vi "CRIOUI.vi"() -> ()   [LabVIEW 2014, in "PLTarget cRIO.lvclass"]
uses:
  PLTarget cRIO.lvclass
  <vilib>/NI/Tag Bus Module Framework/root configuration/Target Types.ctl
  <vilib>/NI/Configuration Framework/Node/NodeRef.ctl
  <vilib>/NI/Configuration Framework/Node/NISE_CEF_Node.lvclass
  <vilib>/NI/AMC/Message Queue.ctl
  <vilib>/NI/AMC/Message.ctl
  <vilib>/NI/Tools/Keyed Array/KeyedArray.ctl
  <vilib>/NI/Configuration Framework/Node/UserEventRef.ctl
  <vilib>/NI/Configuration Framework/Controls/EventCluster.ctl
  <vilib>/NI/Configuration Framework/Node/RefreshUIEvent.ctl
  <vilib>/NI/Configuration Framework/Node/CacheState.ctl
  <vilib>/NI/Configuration Framework/Node/StopEvent.ctl
  <vilib>/NI/Configuration Framework/Node/NodeChangeEvent.ctl
  Configuration Editor/subVIs/Additional Files Array.ctl
  Configuration Editor/Classes/TBM Configuration Node/deployment configuration.ctl
  <vilib>/Utility/miscctls.llb/LVPositionTypeDef.ctl
  Configuration Editor/Classes/Targets/Targets.lvclass/Targets.ctl
  PLTarget cRIO.lvclass/PLTarget cRIO.ctl
  Framework Configuration Classes/target configuration/PL_Target Configuration.lvclass/PL_Target Configuration.ctl
  <vilib>/NI/Configuration Framework/serializable node/NISE_CEF_serializable node.lvclass
  <vilib>/NI/Tag Bus Module Framework/root configuration/TBM configuration.lvclass
  Configuration Editor/Classes/Targets/Write additional files.vi
  Configuration Editor/Classes/Targets/Read additional files.vi
  <vilib>/NI/Configuration Framework/serializable configuration/set alias.vi
  <vilib>/NI/Configuration Framework/serializable configuration/get alias.vi
  <vilib>/NI/Configuration Framework/serializable configuration/NISE_CEF_serializable configuration.lvclass
  Framework Configuration Classes/target configuration/PL_Target Configuration.lvclass
  Configuration Editor/Classes/Targets/Targets.lvclass
  <vilib>/NI/DCAF UI Toolkit/Controls/DCAF UI Elements.lvlib
  <vilib>/NI/Tools/Keyed Array/Tools_KeyedArray.lvlib
  <vilib>/NI/AMC/AMC.lvlib
  <vilib>/NI/Configuration Framework/NISE_CEF_TreeControl.lvlib
  Configuration Editor/Classes/TBM Configuration Node/TBM Configuration Node.lvclass
panel:
  in  "Top Level Tab Control":enum32{"Configuration", "Additional Files"}(tab)
  in  "Target Type":T1=enum."Linux RT ARM"
  in  "IP":string
  in  "Name":string
  in  "Includes file path":path
  in  "path to deploy on target relative to root (c:\\ or /home/lvuser/)":path
  in  "generate includes file":bool
  in  "load bitfile":bool
  in  "RIO FPGA":string="RIO0"
  in  "bitfile path on target relative to root (c:\\ or /home/lvuser/)":path
  in  "Local Bitfile Path":path
  in  "Additional Files":T2
  in  "node change":T4
  in  "stop event":T5
  in  "cache state":T6
  in  "refresh UI":T7
  in  "open fp?":bool=TRUE
  in  "user event":T8
  in  "main queue":T9
  in  "node ref":T10
  # "Target Information"
  # "Deployment Settings"
  # "FPGA Settings"
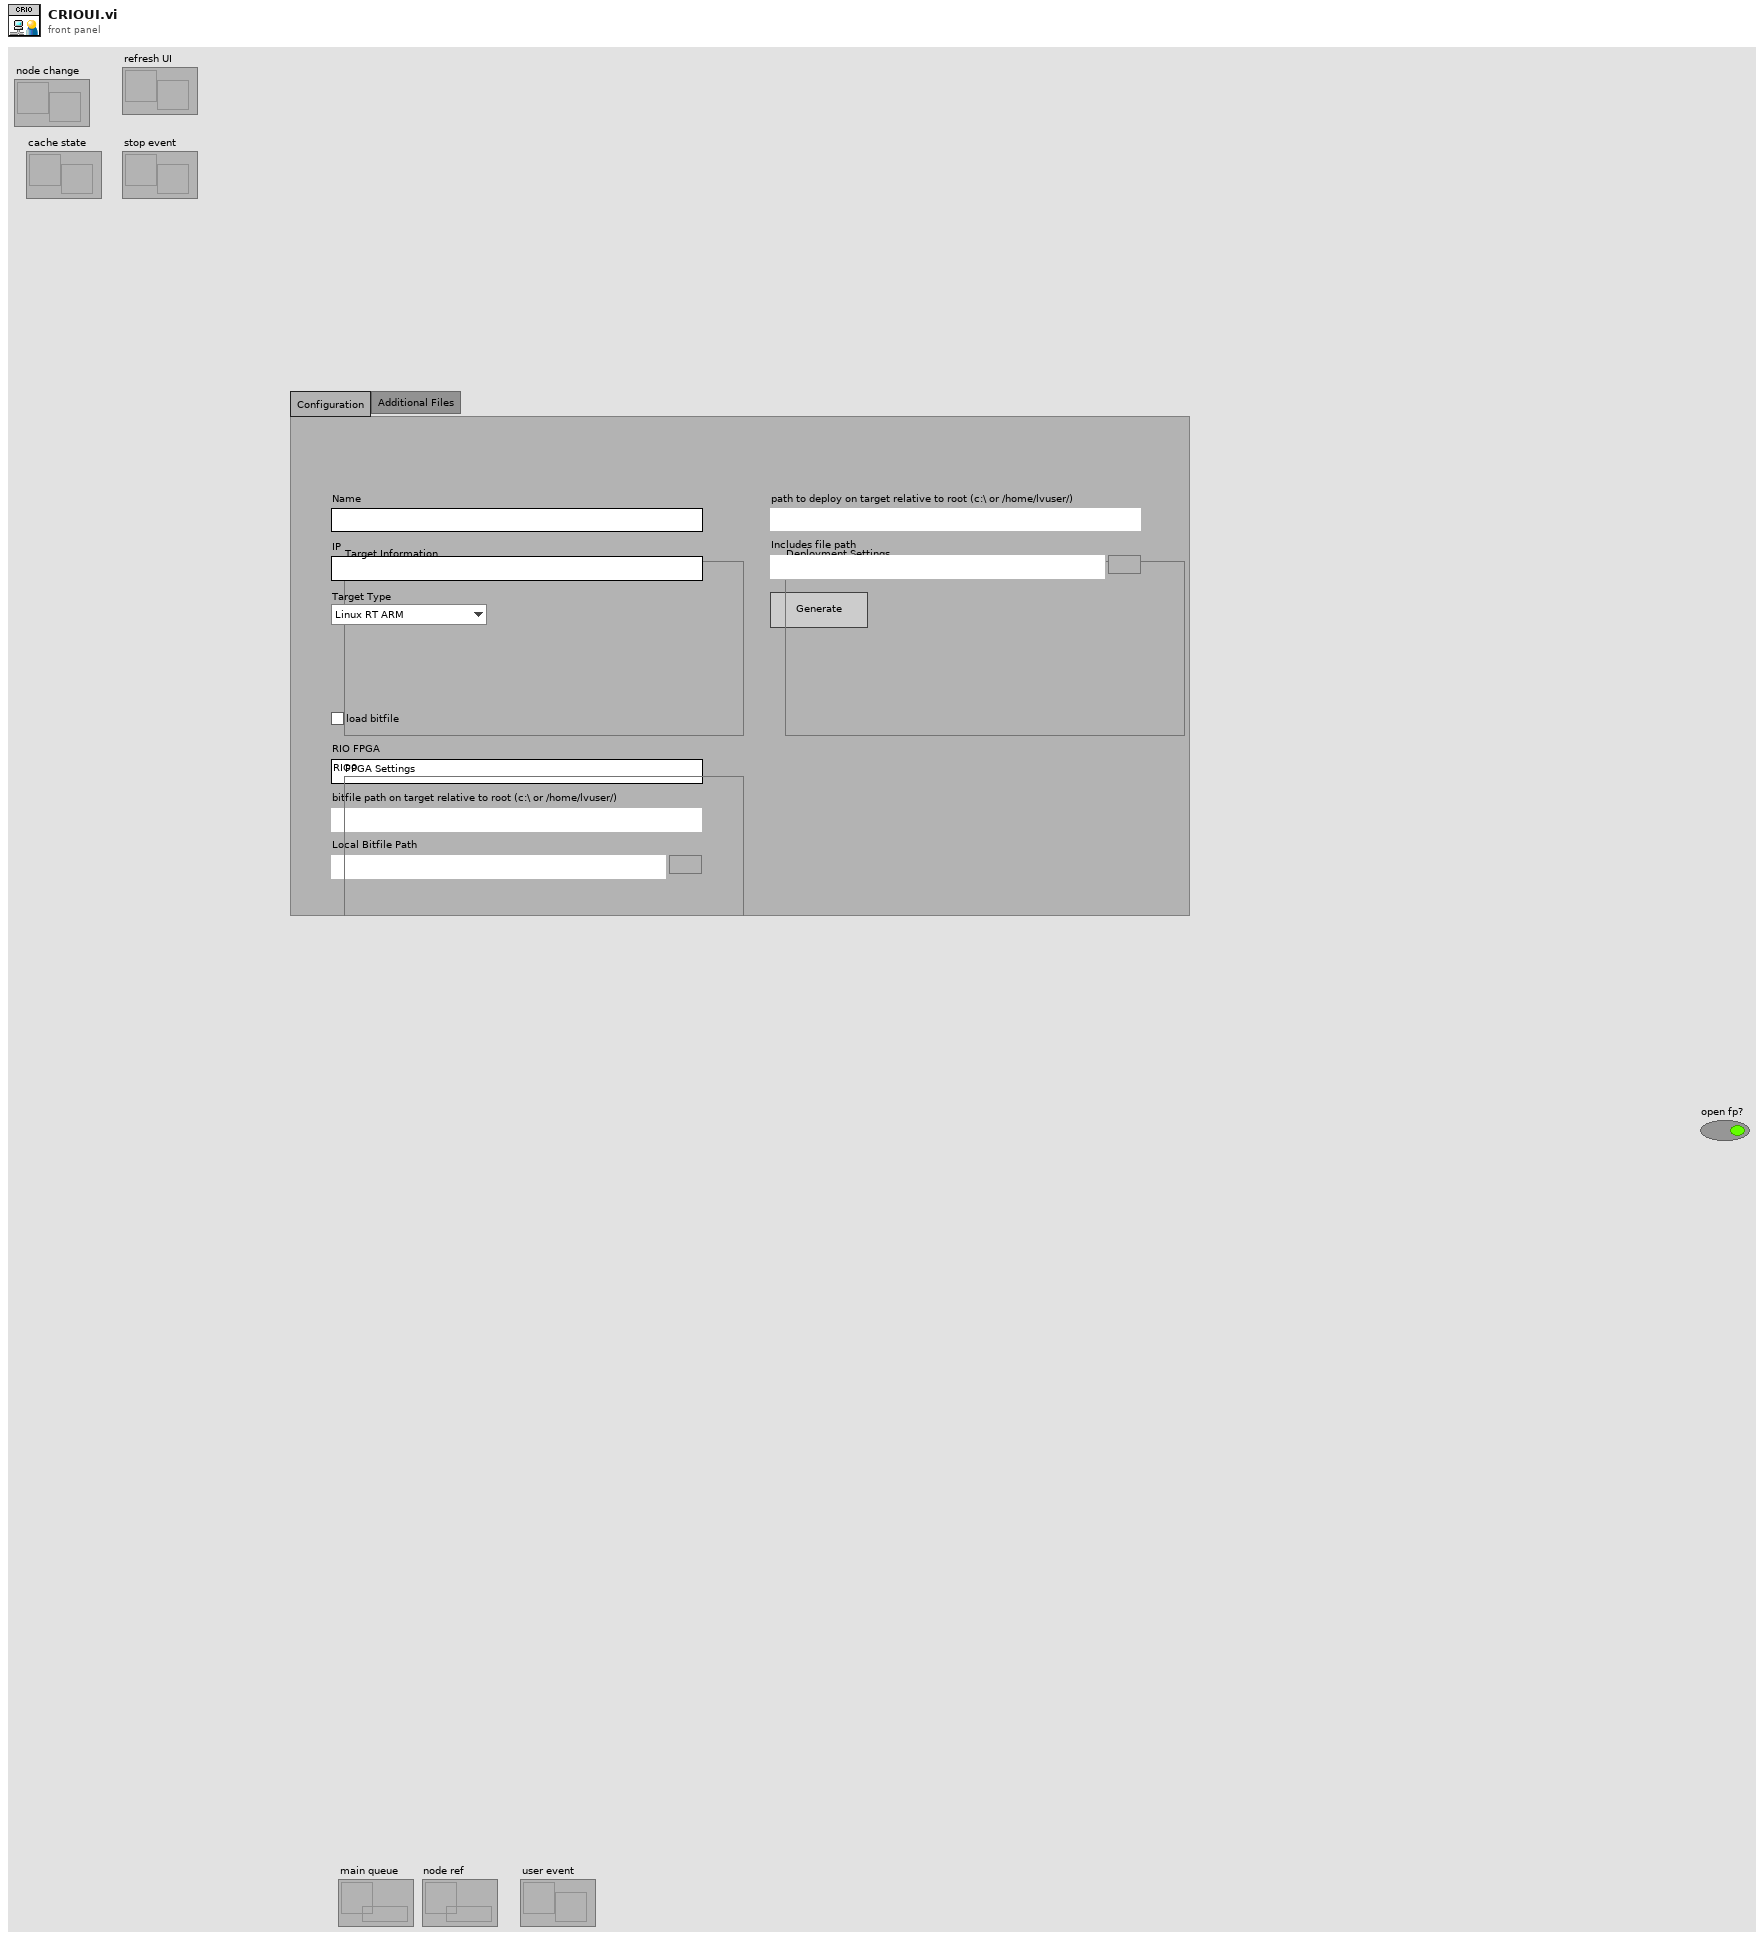
[diagram p1: front panel]
types:
  T1 = typedef "TBM configuration.lvclass/Target Types.ctl" = enum16{"Windows", "Mac", "Linux", "Linux RT ARM", "VxWorks", "Pharlap", "Other", "Linux RT x64"}
  T2 = typedef "Additional Files Array.ctl" = T3[]
  T3 = typedef "PL Framework Configuration Tool.lvlib/TBM Configuration Node.lvclass/deployment configuration.ctl" = cluster{"local path":path, "remote path (relative to root)":path}
  T4 = typedef "NISE_CEF_Node.lvclass/NodeChangeEvent.ctl" = refnum<user-event>
  T5 = typedef "NISE_CEF_Node.lvclass/StopEvent.ctl" = refnum<user-event>
  T6 = typedef "NISE_CEF_Node.lvclass/CacheState.ctl" = refnum<user-event>
  T7 = typedef "NISE_CEF_Node.lvclass/RefreshUIEvent.ctl" = refnum<user-event>
  T8 = typedef "NISE_CEF_Node.lvclass/UserEventRef.ctl" = refnum<user-event>
  T9 = typedef "AMC.lvlib/Message Queue.ctl" = refnum<queue>
  T10 = typedef "NISE_CEF_Node.lvclass/NodeRef.ctl" = refnum<data-value>
  T11 = typedef "LVPositionTypeDef.ctl" = cluster{"Left":i32, "Top":i32}
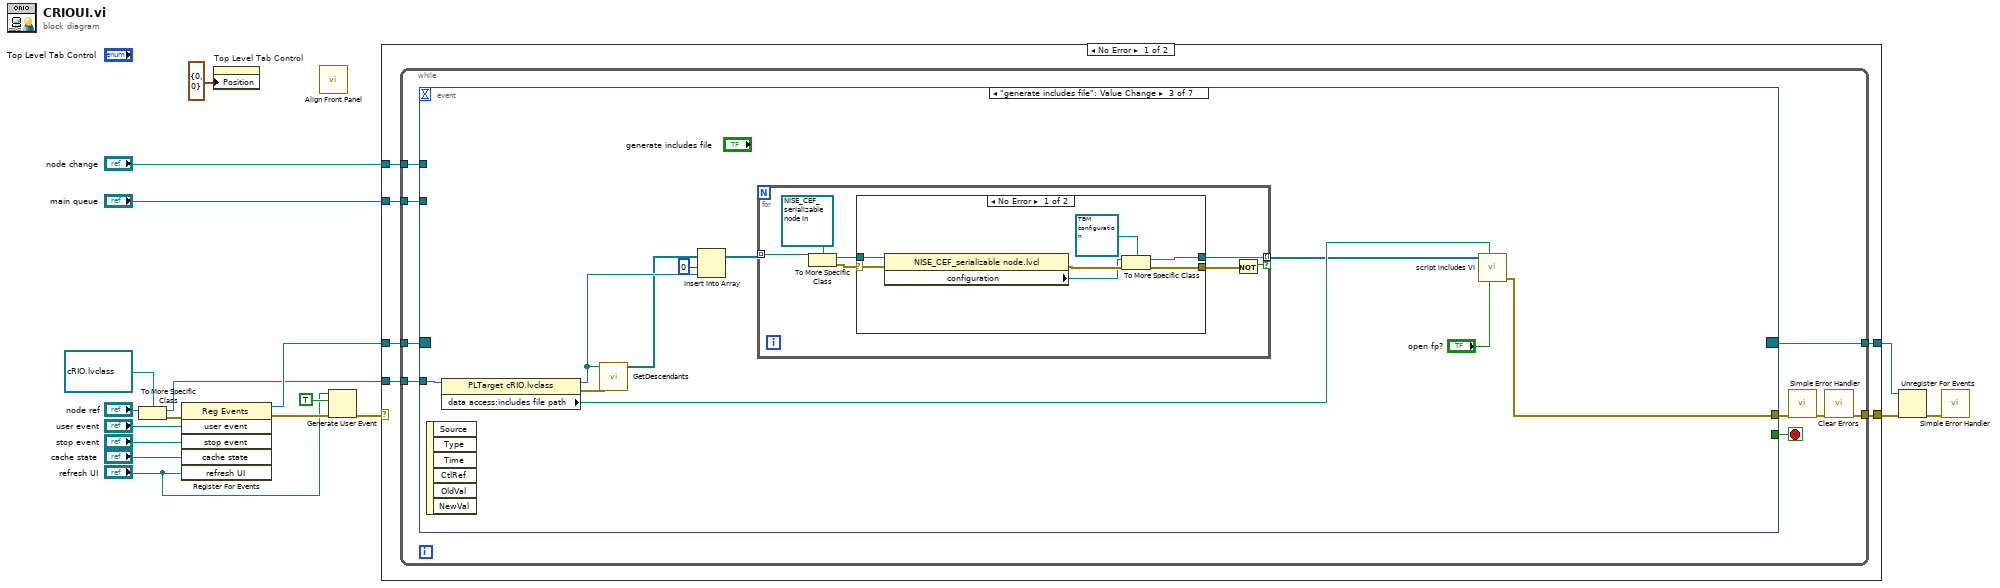
[diagram p0: block diagram]
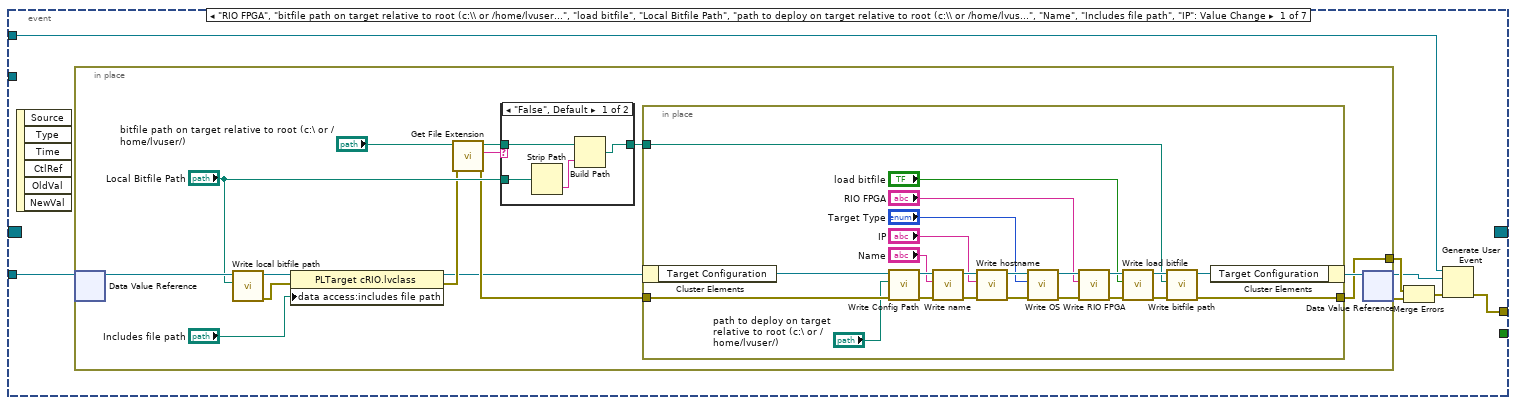
[diagram p2: hidden frame]
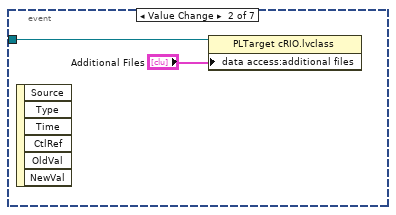
[diagram p4: hidden frame]
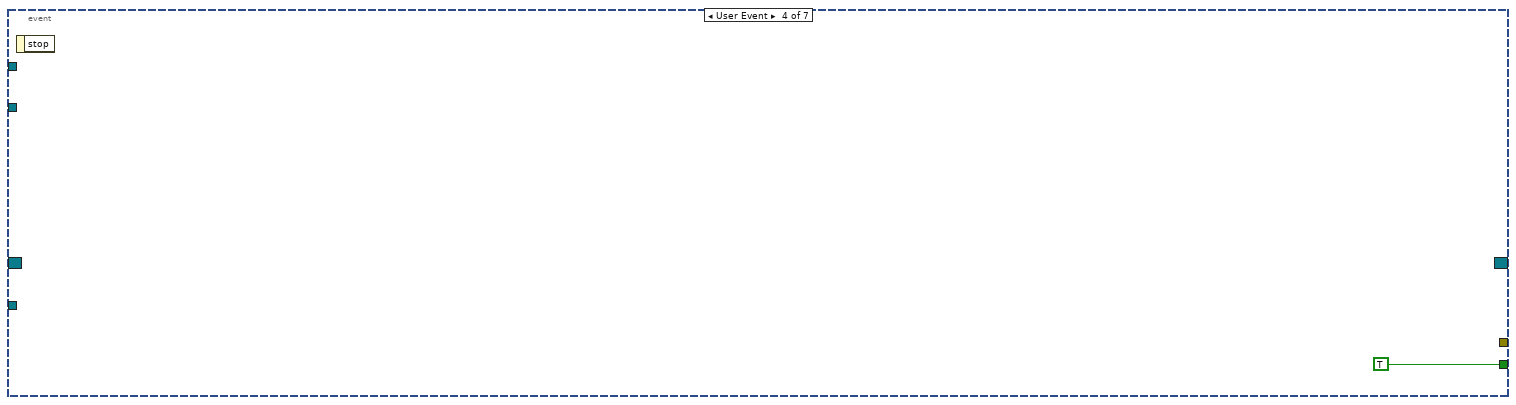
[diagram p6: hidden frame]
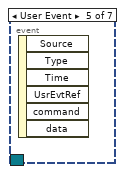
[diagram p7: hidden frame]
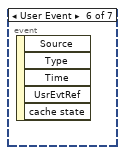
[diagram p8: hidden frame]
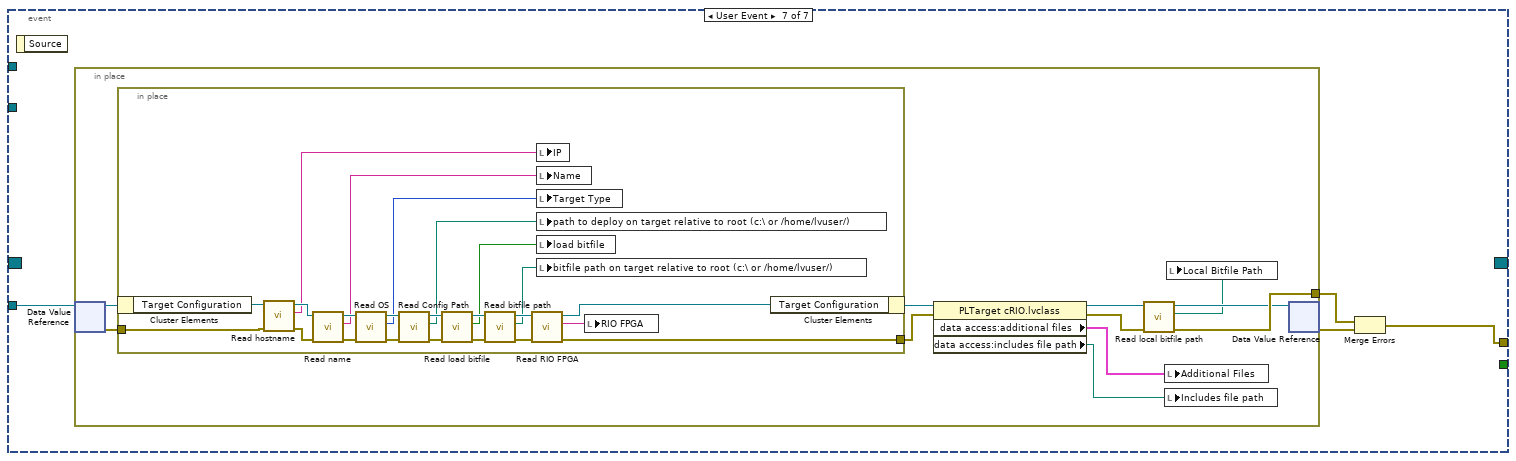
[diagram p9: hidden frame]
diagram:
  n1 = To More Specific Class(target class=refnum<data-value> refnum ("data value reference"), reference="node ref") -> (specific class reference=w6:refnum<data-value>, error out=w7:errorcluster)  [unwired: 1 in]
  n2 = register-events(error in=w7, "user event", "stop event", "cache state", "refresh UI") -> (reference out=w16:refnum<event-registration>, error out=w13:errorcluster)  [unwired: 1 in]
  n3 = property on="Top Level Tab Control" class="TabCtl (strict)"("Position"=T11 {"Left"=0, "Top"=0}) -> ()  [unwired: 2 in, 2 out]
  n4 = call <vilib>:"Align Front Panel.vi"() -> ()  [unwired: 10 in, 2 out]
  n5 = Generate User Event(user event="refresh UI", event data cluster=TRUE ("event data"), error in=w13) -> (error out=w8:errorcluster)  [unwired: 1 in, 1 out]
  n6 = case shown="No Error" w8 {
    selector: w8 -> [_ w149]
    tunnel: w6 -> [w24 _]
    tunnel: "main queue" -> [w23 _]
    tunnel: w16 -> [w22 w150]
    tunnel: [w21 w150] -> w15
    tunnel: [w20 w149] -> w14
    tunnel: "node change" -> [w19 _]
    frame No Error {
      n7 = while {
        tunnel: w24 -> [w33]
        tunnel: w23 -> [w32]
        tunnel: w22 -> [w31]
        tunnel: [w30] -> w21
        tunnel: [w26] -> w20
        tunnel: w19 -> [w25]
        stop <- w29 stop-if-true
        n8 = event shown="[2] \"generate includes file\": Value Change" {
          selector: w31 -> [_ _ _ _ _ _ _]
          dyn-events: [_ _ _ _ _ _ _] -> w30
          timeout: _ -> [_ _ _ _ _ _ _]
          tunnel: w33 -> [w40 w84 w94 _ _ _ w114]
          tunnel: w32 -> [_ _ _ _ _ _ _]
          tunnel: [_ _ _ TRUE _ _ _] -> w29
          tunnel: [w38 _ w91 _ _ _ w112] -> w28
          tunnel: w25 -> [w37 _ _ _ _ _ _]
          event "RIO FPGA", "bitfile path on target relative to root (c:\\ or /home/lvuser/)", "load bitfile", "Local Bitfile Path", "path to deploy on target relative to root (c:\\ or /home/lvuser/)", "Name", "Includes file path", "IP": Value Change {
            n9 = event-data() -> ()  [unwired: 1 in, 6 out]
            n10 = in-place {
              in-place-border: [w53] -> w39
              n11 = in-place-dvr #1(w40) -> (w52:refnum<class "PLTarget cRIO.lvclass">)  [unwired: 1 out]
              n12 = call "Write local bitfile path.vi"("bitfile path"="Local Bitfile Path", "Targets in"=w52) -> ("error out"=w46:errorcluster, "Targets out"=w43:refnum<class "PLTarget cRIO.lvclass">)  [unwired: 8 in]
              n13 = property class="PLTarget cRIO.lvclass"(reference=w43, error in=w46, "data access:includes file path"="Includes file path") -> (reference out=w42:refnum<class "PLTarget cRIO.lvclass">, error out=w44:errorcluster)
              n14 = call <vilib>:"Get File Extension.vi"("error in (no error)"=w44, "file"="bitfile path on target relative to root (c:\\ or /home/lvuser/)") -> ("error out"=w45:errorcluster, "lowercase file extension"=w50:string, "dup file"=w48:path)  [unwired: 6 in, 1 out]
              n15 = case shown="\"False\", Default" w50 {
                tunnel: [w57 w59] -> w49
                tunnel: w48 -> [w58 w59]
                tunnel: "Local Bitfile Path" -> [w55 _]
                frame "False", Default {
                  n16 = Strip Path(path=w55) -> (name=w56:string)  [unwired: 1 out]
                  n17 = Build Path(base path=w58, name or relative path=w56) -> (appended path=w57:path)
                }
                frame "lvbit", "lvbitx" {
                }
              }
              n18 = in-place {
                in-place-border: w45 -> [w68]
                in-place-border: [w67] -> w53
                in-place-border: w49 -> [w64]
                n19 = in-place-cluster #2(w42) -> ("Target Configuration"=w82:refnum<class "PL_Target Configuration.lvclass">)
                n20 = call "Write Config Path.vi"("error in"=w68, "Config Path"="path to deploy on target relative to root (c:\\ or /home/lvuser/)", "PL_Local Target Configuration in"=w82) -> ("error out"=w72:errorcluster, "PL_Local Target Configuration out"=w81:refnum<class "PL_Target Configuration.lvclass">)  [unwired: 7 in]
                n21 = call "Write name.vi"("error in"=w72, "name"="Name", "PL_Local Target Configuration in"=w81) -> ("error out"=w71:errorcluster, "PL_Local Target Configuration out"=w80:refnum<class "PL_Target Configuration.lvclass">)  [unwired: 7 in]
                n22 = call "Write hostname.vi"("error in"=w71, "hostname"="IP", "PL_Target Configuration in"=w80) -> ("error out"=w70:errorcluster, "PL_Target Configuration out"=w79:refnum<class "PL_Target Configuration.lvclass">)  [unwired: 7 in]
                n23 = call "Write OS.vi"("error in"=w70, "Target Types"="Target Type", "PL_Target Configuration in"=w79) -> ("error out"=w69:errorcluster, "PL_Target Configuration out"=w74:refnum<class "PL_Target Configuration.lvclass">)  [unwired: 7 in]
                n24 = call "Write RIO FPGA.vi"("error in"=w69, "RIO FPGA"="RIO FPGA", "PL_Target Configuration in"=w74) -> ("error out"=w76:errorcluster, "PL_Target Configuration out"=w75:refnum<class "PL_Target Configuration.lvclass">)  [unwired: 7 in]
                n25 = call "Write load bitfile.vi"("error in"=w76, "load bitfile"="load bitfile", "PL_Target Configuration in"=w75) -> ("error out"=w78:errorcluster, "PL_Target Configuration out"=w77:refnum<class "PL_Target Configuration.lvclass">)  [unwired: 7 in]
                n26 = call "Write bitfile path.vi"("error in"=w78, "bitfile path"=w64, "PL_Target Configuration in"=w77) -> ("error out"=w67:errorcluster, "PL_Target Configuration out"=w73:refnum<class "PL_Target Configuration.lvclass">)  [unwired: 7 in]
                n27 = in-place-cluster #2("Target Configuration"=w73) -> (w54:refnum<class "PLTarget cRIO.lvclass">)
              }
              n28 = in-place-dvr #1(w54) -> (w36:refnum<data-value>, w34:errorcluster)
            }
            n29 = Merge Errors(w39, w34) -> (w35:errorcluster)
            n30 = Generate User Event(user event=w37, event data cluster=w36, error in=w35) -> (error out=w38:errorcluster)  [unwired: 1 in, 1 out]
          }
          event Value Change {
            n31 = event-data() -> ()  [unwired: 1 in, 6 out]
            n32 = property class="PLTarget cRIO.lvclass"(reference=w84, "data access:additional files"="Additional Files") -> ()  [unwired: 1 in, 2 out]
          }
          event "generate includes file": Value Change {
            n33 = event-data() -> ()  [unwired: 1 in, 6 out]
            n34 = property class="PLTarget cRIO.lvclass"(reference=w94) -> (reference out=w88:refnum<data-value>, error out=w90:errorcluster, "data access:includes file path"=w92:path)  [unwired: 1 in]
            n35 = call <vilib>:"GetDescendants.vi"("error in"=w90, "node in"=w88) -> ("descendants"=w87:refnum<data-value>[])  [unwired: 8 in, 1 out]
            n36 = Insert Into Array(array=w87, index=0, new element=w88) -> (w86:refnum<data-value>[])
            n37 = for {
              tunnel: w86 -> [w101] mode=indexing
              tunnel: [w97] -> w89 mode=indexing if=w95
              n38 = To More Specific Class(target class=refnum<data-value> refnum, reference=w101) -> (specific class reference=w98:refnum<data-value>, error out=w99:errorcluster)  [unwired: 1 in]
              n39 = case shown="No Error" w99 {
                selector: w99 -> [w107 w109]
                tunnel: w98 -> [w108 _]
                tunnel: [w102 _] -> w97
                tunnel: [w105 w109] -> w96
                frame No Error {
                  n40 = property class="NISE_CEF_serializable node.lvcl"(reference=w108, error in=w107) -> (error out=w106:errorcluster, "configuration"=w104:refnum<class "NISE_CEF_serializable configuration.lvclass">)  [unwired: 1 out]
                  n41 = To More Specific Class(target class=refnum<class "TBM configuration.lvclass"> refnum ("configuration"), reference=w104, error in=w106) -> (specific class reference=w102:refnum<class "TBM configuration.lvclass">, error out=w105:errorcluster)
                }
                frame Error {
                }
              }
              n42 = Not(x=w96) -> (.not. x?=w95:bool)
            }
            n43 = call "script includes VI.vi"("open fp?"="open fp?", "vi path (blank=new)"=w92, "cfg objects"=w89) -> ("error out"=w91:errorcluster)  [unwired: 8 in]
          }
          event User Event {
            n44 = event-data() -> ()  [unwired: 1 in, 1 out]
          }
          event User Event {
            n45 = event-data() -> ()  [unwired: 1 in, 6 out]
          }
          event User Event {
            n46 = event-data() -> ()  [unwired: 1 in, 5 out]
          }
          event User Event {
            n47 = event-data() -> ()  [unwired: 1 in, 1 out]
            n48 = in-place {
              in-place-border: [w122] -> w111
              n49 = in-place-dvr #3(w114) -> (w125:refnum<class "PLTarget cRIO.lvclass">, w124:errorcluster)
              n50 = in-place {
                in-place-border: w124 -> [w134]
                in-place-border: [w133] -> w123
                n51 = in-place-cluster #4(w125) -> ("Target Configuration"=w146:refnum<class "PL_Target Configuration.lvclass">)
                n52 = call "Read hostname.vi"("error in"=w134, "PL_Target Configuration in"=w146) -> ("error out"=w144:errorcluster, "hostname"=w129:string, "PL_Target Configuration out"=w147:refnum<class "PL_Target Configuration.lvclass">)  [unwired: 7 in]
                n53 = call "Read name.vi"("error in"=w144, "PL_Local Target Configuration in"=w147) -> ("error out"=w143:errorcluster, "name"=w128:string, "PL_Local Target Configuration out"=w148:refnum<class "PL_Target Configuration.lvclass">)  [unwired: 7 in]
                n54 = call "Read OS.vi"("error in"=w143, "PL_Target Configuration in"=w148) -> ("error out"=w142:errorcluster, "Target Types"=w127:T1, "PL_Target Configuration out"=w145:refnum<class "PL_Target Configuration.lvclass">)  [unwired: 7 in]
                n55 = call "Read Config Path.vi"("error in"=w142, "PL_Local Target Configuration in"=w145) -> ("error out"=w135:errorcluster, "Config Path"=w126:path, "PL_Local Target Configuration out"=w136:refnum<class "PL_Target Configuration.lvclass">)  [unwired: 7 in]
                n56 = call "Read load bitfile.vi"("error in"=w135, "PL_Target Configuration in"=w136) -> ("error out"=w139:errorcluster, "load bitfile"=w130:bool, "PL_Target Configuration out"=w138:refnum<class "PL_Target Configuration.lvclass">)  [unwired: 7 in]
                n57 = call "Read bitfile path.vi"("error in"=w139, "PL_Target Configuration in"=w138) -> ("error out"=w141:errorcluster, "bitfile path"=w131:path, "PL_Target Configuration out"=w140:refnum<class "PL_Target Configuration.lvclass">)  [unwired: 7 in]
                n58 = call "Read RIO FPGA.vi"("error in"=w141, "PL_Target Configuration in"=w140) -> ("error out"=w133:errorcluster, "RIO FPGA"=w132:string, "PL_Target Configuration out"=w137:refnum<class "PL_Target Configuration.lvclass">)  [unwired: 7 in]
                n59 = local write "IP"(w129) -> ()
                n60 = local write "Name"(w128) -> ()
                n61 = local write "Target Type"(w127) -> ()
                n62 = local write "path to deploy on target relative to root (c:\\ or /home/lvuser/)"(w126) -> ()
                n63 = local write "load bitfile"(w130) -> ()
                n64 = local write "bitfile path on target relative to root (c:\\ or /home/lvuser/)"(w131) -> ()
                n65 = local write "RIO FPGA"(w132) -> ()
                n66 = in-place-cluster #4("Target Configuration"=w137) -> (w118:refnum<class "PLTarget cRIO.lvclass">)
              }
              n67 = property class="PLTarget cRIO.lvclass"(reference=w118, error in=w123) -> (reference out=w117:refnum<class "PLTarget cRIO.lvclass">, error out=w119:errorcluster, "data access:additional files"=w115:T3[], "data access:includes file path"=w116:path)
              n68 = call "Read local bitfile path.vi"("error in"=w119, "Targets in"=w117) -> ("error out"=w122:errorcluster, "bitfile path"=w120:path, "Targets out"=w121:refnum<class "PLTarget cRIO.lvclass">)  [unwired: 7 in]
              n69 = local write "Additional Files"(w115) -> ()
              n70 = local write "Includes file path"(w116) -> ()
              n71 = local write "Local Bitfile Path"(w120) -> ()
              n72 = in-place-dvr #3(w121) -> (w113:errorcluster)  [unwired: 1 out]
            }
            n73 = Merge Errors(w111, w113) -> (w112:errorcluster)
          }
        }
        n74 = call <vilib>:"Simple Error Handler.vi"("error in (no error)"=w28) -> ("error out"=w27:errorcluster)  [unwired: 4 in, 4 out]
        n75 = call <vilib>:"Clear Errors.vi"("error in (no error)"=w27) -> ("error out"=w26:errorcluster)  [unwired: 5 in, 1 out]
      }
    }
    frame Error {
    }
  }
  n76 = Unregister For Events(event registration refnum=w15, error in=w14) -> (error out=w5:errorcluster)
  n77 = call <vilib>:"Simple Error Handler.vi"("error in (no error)"=w5) -> ()  [unwired: 4 in, 5 out]
